vi "region analysis.vi"(8 "MAX Duration time(s)":dbl=0.01 format="%#_13g", 9 "MAX E and S time(s)":dbl=0.01 format="%#_13g", 11 "S Table C1":T7) -> (0 "All Signal Intensity Histogram":T4(graph), 1 "D-I Graph":T5(graph), 2 "Duration Graph":cluster{i32[], dbl[]}(graph), 3 "STD Graph":T6(graph), 4 "Burst Array":T1, 5 "Burst Time Profile":cluster{i32[], "SDS":dbl[]}[](graph), 6 "Under D array":T2, 7 "Region Info":T3)   [LabVIEW 2018]
uses:
  <vilib>/Analysis/NI_AALBase.lvlib
  <vilib>/gmath/NI_Gmath.lvlib
panel:
  out "R S IDX":i32[](array[numeric])
  out "under D BL":dbl[](array[numeric])
  out "Burst A":cluster{"Total Burst (s)":dbl, "B time (%)":dbl}
  out "Burst Region (n)":i32
  out "SDS":dbl[](array[numeric])
  out "SN (%)":dbl
  out "mean":dbl caption="Mean (pA)" format="%0.2f"
  out "Signal (n)":i32
  out "spread value":dbl caption="STD (pA)"
  out "Burst Signal Intensity Histogram":T4(graph)
  out "I underD0.01s":dbl[](array[numeric])
  out "Burst (%)":dbl
  out "Burst S (n)":i32
  out "under D 0.01s":dbl[](array[numeric])
  in  "+/- Point":i32=2000
  out "kurtosis":dbl caption="尖度"
  out "skewness":dbl caption="歪度"
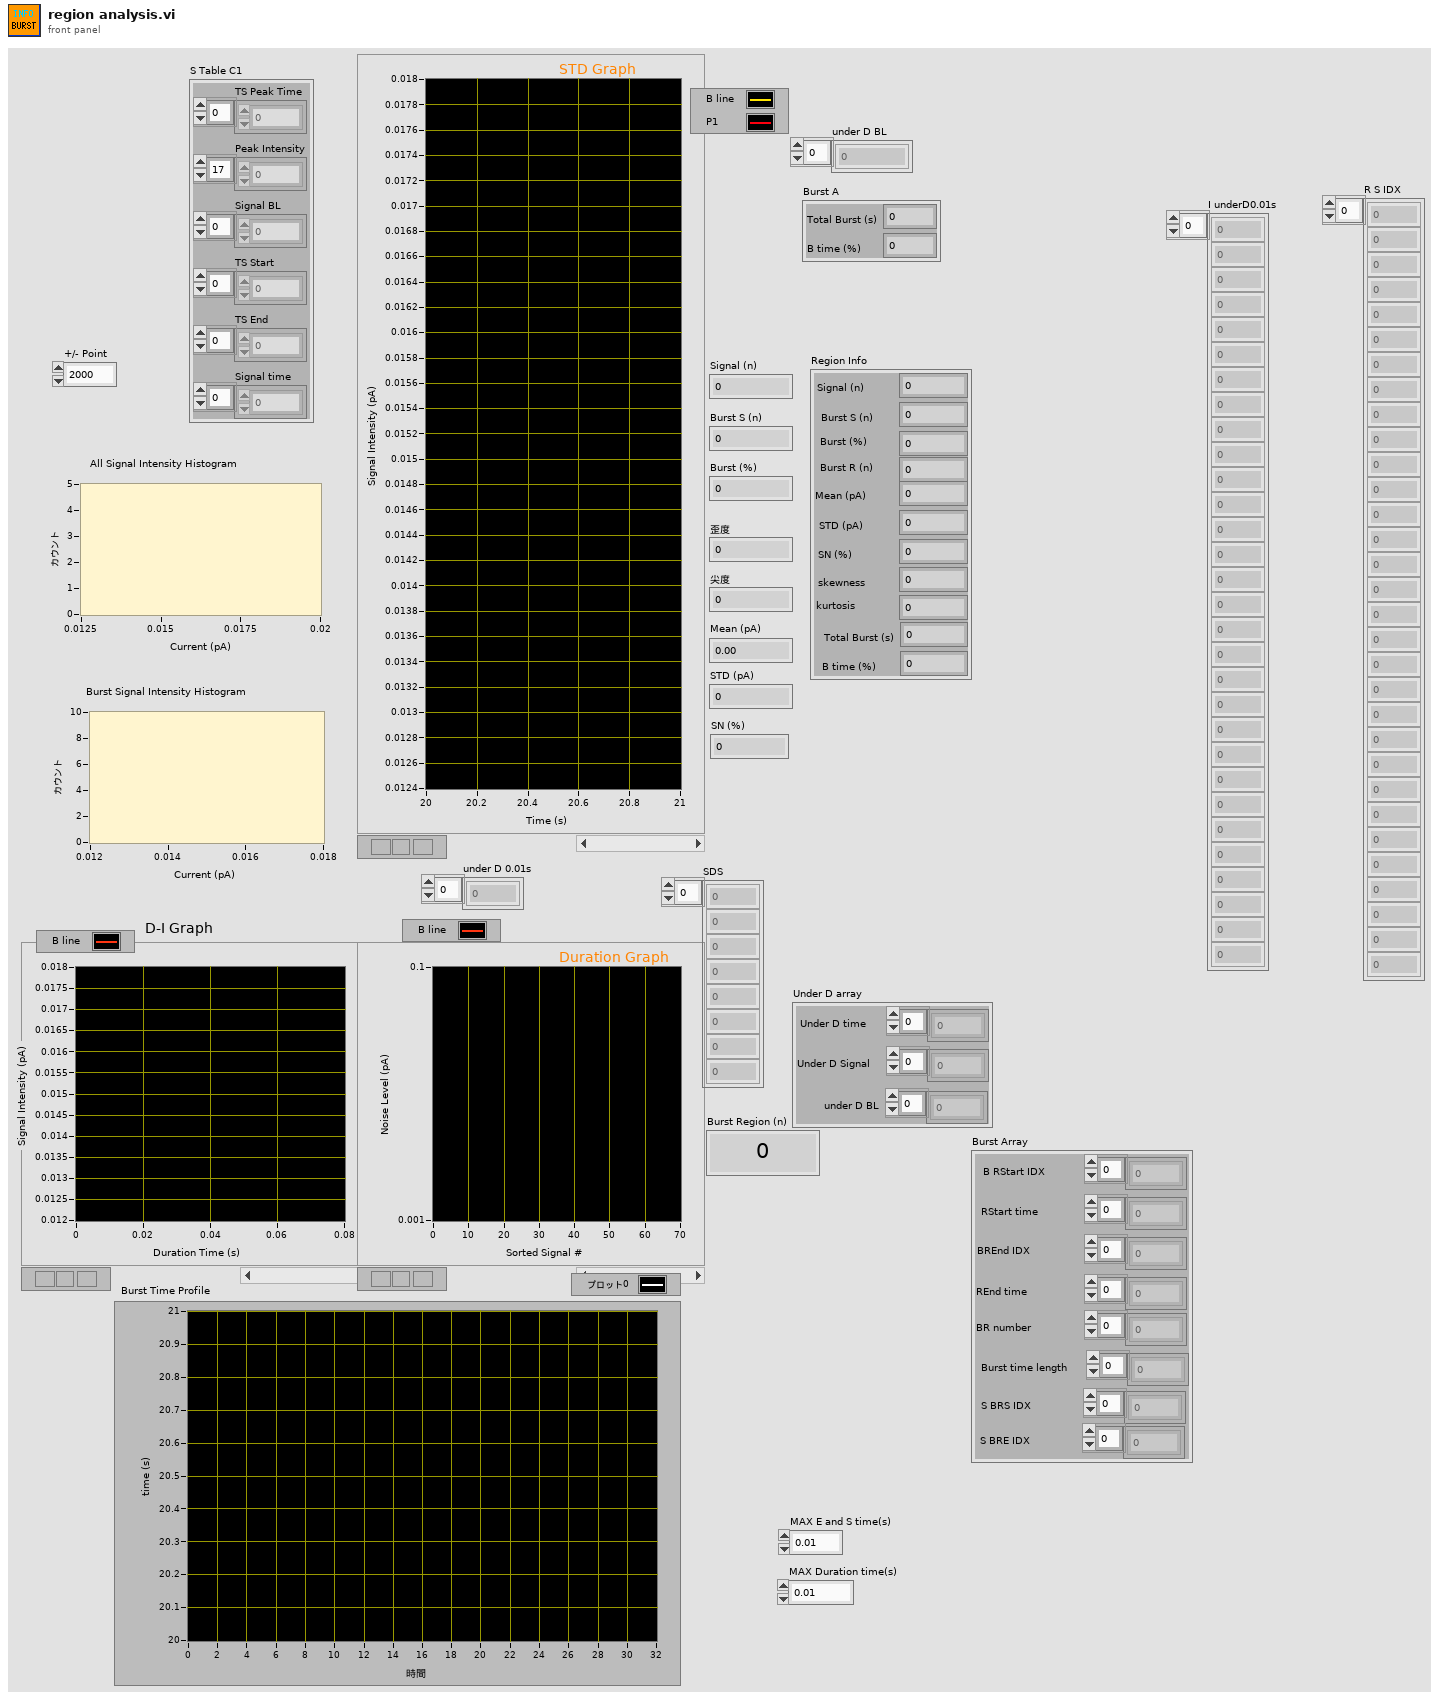
[diagram p1: front panel]
types:
  T1 = cluster{"B RStart IDX":i32[], "RStart time":dbl[], "BREnd IDX":i32[], "REnd time":dbl[], "BR number":dbl[], "Burst time length":dbl[], "S BRS IDX":i32[], "S BRE IDX":i32[]}
  T2 = cluster{"Under D time":dbl[], "Under D Signal":dbl[], "under D BL":dbl[]}
  T3 = cluster{"Signal (n)":i32, "Burst S (n)":i32, "Burst (%)":dbl, "Burst R (n)":dbl, "Mean (pA)":dbl, "STD (pA)":dbl, "SN (%)":dbl, "skewness":dbl, "kurtosis":dbl, "Total Burst (s)":dbl, "B time (%)":dbl}
  T4 = cluster{"X Values":dbl[], "Histogram: h(x)":i32[]}
  T5 = cluster{"TS Start":dbl[], "Peak Intensity":dbl[]}
  T6 = cluster{"TS Start":dbl[], "Peak Intensity":dbl[]}[]
  T7 = cluster{"TS Peak Time":dbl[], "Peak Intensity":dbl[], "Signal BL":dbl[], "TS Start":dbl[], "TS End":dbl[], "Signal time":dbl[]}
  T8 = cluster{i32, i32, dbl, "Burst Region (n)":i32, dbl, dbl, dbl, "skewness":dbl, "kurtosis":dbl, "Total Burst (s)":dbl, "B time (%)":dbl}
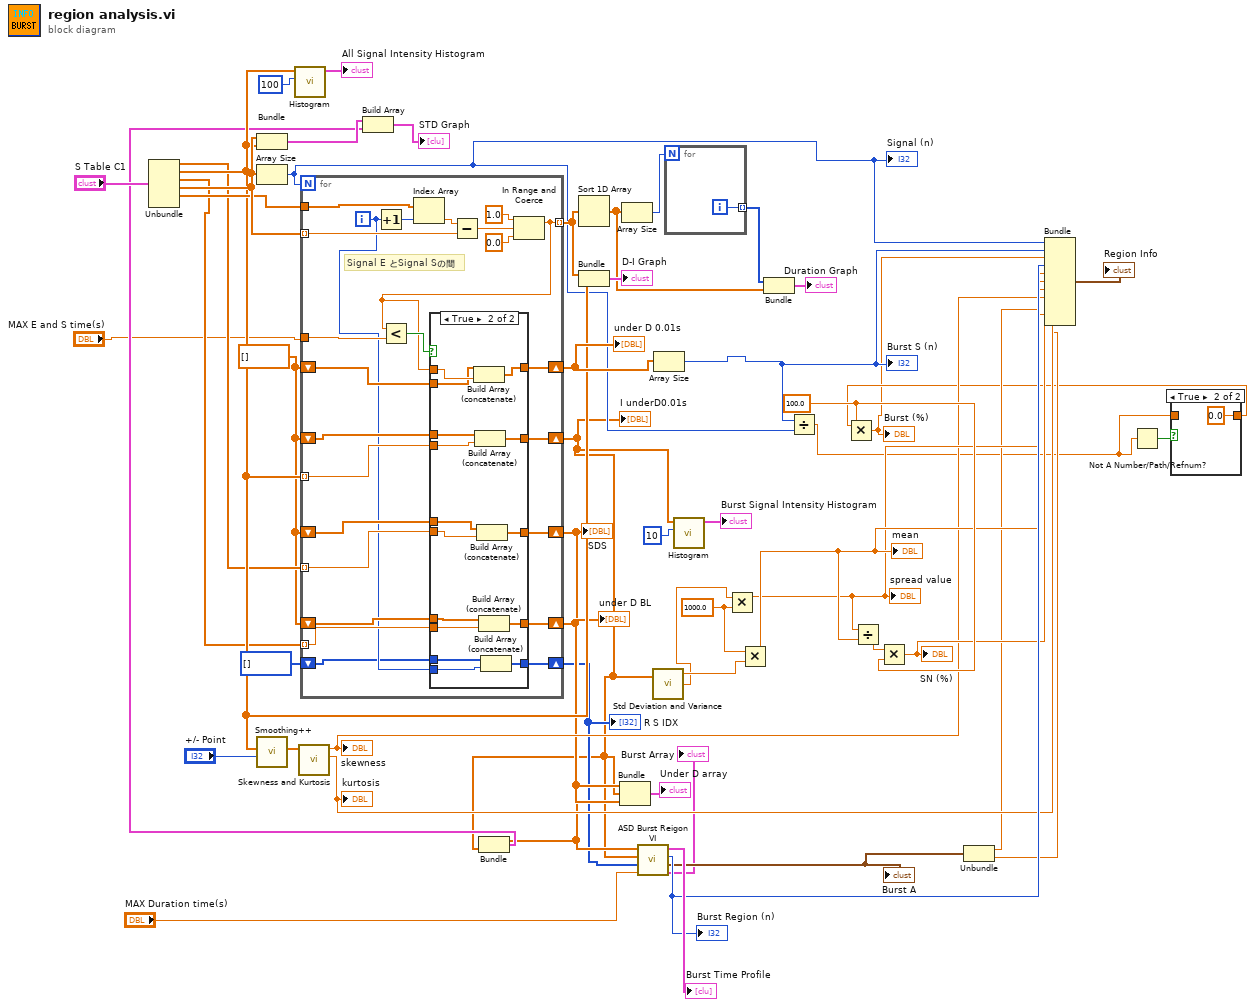
[diagram p0: block diagram]
diagram:
  w36 = 1000.0 ("y")
  w32 = 100.0 ("y")
  w15 = dbl[] []
  n1 = Unbundle("S Table C1") -> ("TS Peak Time"=w34:dbl[], "Peak Intensity"=w40:dbl[], "Signal BL"=w16:dbl[], "TS Start"=w49:dbl[], "TS End"=w48:dbl[])  [unwired: 1 out]
  n2 = Bundle("TS Start"=w49, "Peak Intensity"=w40) -> (w31:T5)  [unwired: 1 in]
  n3 = Array Size(array=w49) -> (size(s)=w27:i32)
  "Signal (n)" <- w27
  n4 = call "Smoothing++.vi"("+/- Point"="+/- Point", "Y in"=w40) -> ("Y out"=w50:dbl[])  [unwired: 9 in]
  n5 = call <vilib>:"Histogram.vi"("intervals"=100, "X"=w40) -> ("Histogram Graph"=→"All Signal Intensity Histogram":T4)  [unwired: 6 in, 3 out]
  n6 = call <vilib>:"Skewness and Kurtosis.vi"("X"=w50) -> ("kurtosis"=w21:dbl, "skewness"=w22:dbl)  [unwired: 8 in, 1 out]
  "skewness" <- w22
  "kurtosis" <- w21
  n7 = for {
    N: w27 -> [_]
    tunnel: w49 -> [w73] mode=indexing
    tunnel: w48 -> [w78]
    tunnel: [w70] -> w42 mode=indexing
    shift-right: [w69] -> w41
    shift-left: w15 -> [w68]
    tunnel: w40 -> [w67] mode=indexing
    shift-right: [w66] -> w2
    shift-left: w15 -> [w65]
    tunnel: w34 -> [w64] mode=indexing
    shift-right: [w63] -> w12
    shift-left: w15 -> [w62]
    tunnel: w16 -> [w61] mode=indexing
    shift-right: [w60] -> w14
    shift-left: w15 -> [w59]
    tunnel: "MAX E and S time(s)" -> [w58]
    shift-right: [w56] -> w3
    shift-left: i32[] [] -> [w55]
    i -> [w57]
    # "Signal E とSignal Sの間"
    n8 = Increment(x=w57) -> (x+1=w76:i32)
    n9 = Index Array(array=w78, index=w76) -> (element=w77:dbl)
    n10 = Subtract(x=w77, y=w73) -> (x-y=w72:dbl)
    n11 = In Range and Coerce(upper limit=1.0 ("上限"), x=w72, lower limit=0.0 ("下限")) -> (coerced(x)=w70:dbl)  [unwired: 1 out]
    n12 = Less?(x=w70, y=w58) -> (x < y?=w71:bool)
    n13 = case shown="True" w71 {
      tunnel: w70 -> [_ w98]
      tunnel: [w83 w97] -> w69
      tunnel: w68 -> [w83 w96]
      tunnel: w67 -> [_ w95]
      tunnel: [w82 w94] -> w66
      tunnel: w65 -> [w82 w93]
      tunnel: w64 -> [_ w92]
      tunnel: [w81 w91] -> w63
      tunnel: w62 -> [w81 w90]
      tunnel: w61 -> [_ w89]
      tunnel: [w80 w88] -> w60
      tunnel: w59 -> [w80 w87]
      tunnel: w57 -> [_ w86]
      tunnel: [w79 w85] -> w56
      tunnel: w55 -> [w79 w84]
      frame False {
      }
      frame True {
        n14 = Build Array (concatenate)(w96, w98) -> (w97:dbl[])
        n15 = Build Array (concatenate)(w93, w95) -> (w94:dbl[])
        n16 = Build Array (concatenate)(w90, w92) -> (w91:dbl[])
        n17 = Build Array (concatenate)(w87, w89) -> (w88:dbl[])
        n18 = Build Array (concatenate)(w84, w86) -> (w85:i32[])
      }
    }
  }
  "under D 0.01s" <- w41
  "I underD0.01s" <- w2
  "SDS" <- w12
  "under D BL" <- w14
  "R S IDX" <- w3
  n19 = Bundle(w12, w2) -> (w13:cluster{dbl[], dbl[]})  [unwired: 1 in]
  n20 = Build Array(w31, w13) -> (→"STD Graph":T6)
  n21 = Sort 1D Array(array=w42) -> (sorted array=w44:dbl[])
  n22 = Bundle(w42, "Peak Intensity"=w40) -> (→"D-I Graph":cluster{dbl[], "Peak Intensity":dbl[]})  [unwired: 1 in]
  n23 = Bundle(w12, w2, w14) -> (→"Under D array":cluster{dbl[], dbl[], dbl[]})  [unwired: 1 in]
  n24 = Array Size(array=w44) -> (size(s)=w45:i32)
  n25 = call "ASD Burst Reigon VI.vi"("MAX Duration time(s)"="MAX Duration time(s)", "R S IDX"=w3, "I underD0.01s"=w2, "SDS"=w12) -> ("Burst Array"=→"Burst Array":T1, "Burst A"=w19:cluster{"Total Burst (s)":dbl, "B time (%)":dbl}, "Burst Region (n)"=w26:i32, "Burst Profile"=→"Burst Time Profile":cluster{i32[], "SDS":dbl[]}[])  [unwired: 4 in]
  "Burst Region (n)" <- w26
  "Burst A" <- w19
  n26 = call <vilib>:"Std Deviation and Variance.vi"("X"=w2) -> ("mean"=w37:dbl, "standard deviation"=w35:dbl)  [unwired: 1 in, 1 out]
  n27 = Array Size(array=w41) -> (size(s)=w11:i32)
  "Burst S (n)" <- w11
  n28 = for {
    N: w45 -> [_]
    tunnel: [w99] -> w43 mode=indexing
    i -> [w99]
  }
  n29 = call <vilib>:"Histogram.vi"("intervals"=10, "X"=w2) -> ("Histogram Graph"=→"Burst Signal Intensity Histogram":T4)  [unwired: 6 in, 3 out]
  n30 = Multiply(x=w35, y=w36) -> (x*y=w24:dbl)
  "spread value" <- w24
  n31 = Multiply(x=w36, y=w37) -> (x*y=w25:dbl)
  "mean" <- w25
  n32 = Bundle(w43, w44) -> (→"Duration Graph":cluster{i32[], dbl[]})  [unwired: 1 in]
  n33 = Divide(x=w11, y=w27) -> (x/y=w9:dbl)
  n34 = Divide(x=w24, y=w25) -> (x/y=w33:dbl)
  n35 = Multiply(x=w33, y=w32) -> (x*y=w23:dbl)
  "SN (%)" <- w23
  n36 = Unbundle(w19) -> ("Total Burst (s)"=w18:dbl, "B time (%)"=w17:dbl)
  n37 = Not A Number/Path/Refnum?(number/path/refnum=w9) -> (NaN/Path/Refnum?=w10:bool)
  n38 = case shown="True" w10 {
    tunnel: w9 -> [w100 _]
    tunnel: [w100 0.0 ("Latest M/T (um/V)")] -> w8
    frame False {
    }
    frame True {
    }
  }
  n39 = Multiply(x=w8, y=w32) -> (x*y=w7:dbl)
  "Burst (%)" <- w7
  n40 = Bundle(w27, w11, w7, "Burst Region (n)"=w26, w25, w24, w23, "skewness"=w22, "kurtosis"=w21, "Total Burst (s)"=w18, "B time (%)"=w17) -> (→"Region Info":T8)  [unwired: 1 in]
